vi "FileDialogAsynch.vi"(0 "start path":path=path "", 1 "default name":string, 2 "File dialog event":T1, 5 "pattern (all files)":string, 7 "pattern label":string, 9 "selection mode":T2(ring)=enum."new or existing file", 11 "error in":errorcluster, 12 "button label":string, 13 "prompt":string) -> (15 "error out":errorcluster)   [LabVIEW 2025]
uses:
  FileDialogEvent.ctl
  FileDialogResult.ctl
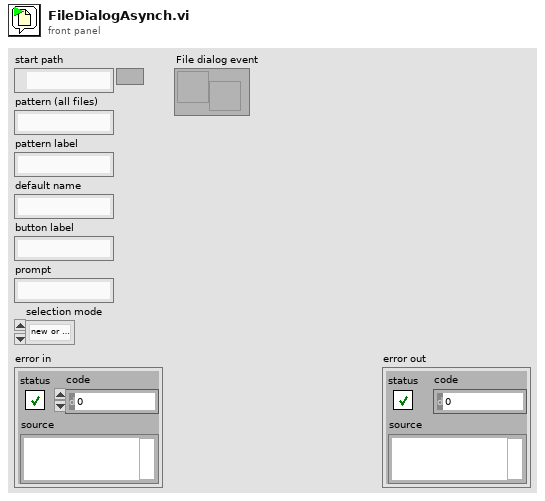
[diagram p1: front panel]
types:
  T1 = typedef "FileDialogEvent.ctl" = refnum<user-event>
  T2 = enum32{"existing file", "new file", "new or existing file", "existing dir", "new dir", "new or existing dir", "existing file (use LLBs)", "new file (use LLBs)", "new or existing file (use LLBs)", "new or existing file or directory (use LLBs)", "existing dir (use LLBs)", "new dir (use LLBs)", "new or existing dir (use LLBs)", "existing file or dir", "new file or dir", "new or existing file or dir", "existing file or dir (use LLBs)", "new file or dir (use LLBs)", "multi-select", "multi-select (use LLBs)"}
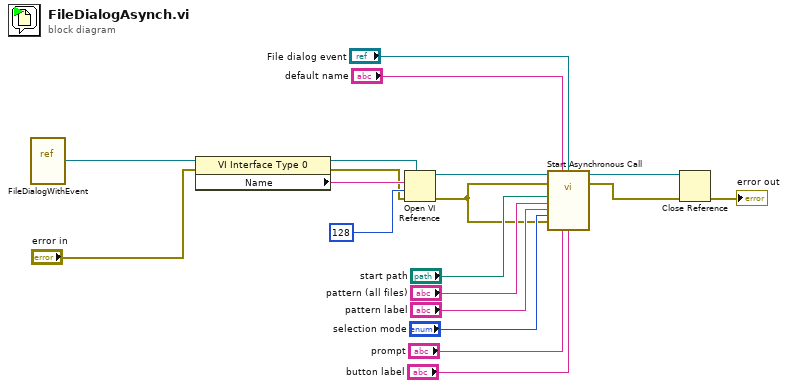
[diagram p0: block diagram]
diagram:
  n1 = vi-ref "FileDialogWithEvent.vi"() -> (w15:refnum<vi>)
  n2 = property class="VI Interface Type 0"(reference=w15, error in="error in") -> (reference out=w1:refnum<vi>, error out=w13:errorcluster, "Name"=w19:string)
  n3 = Open VI Reference(type specifier VI Refnum (for type only)=w1, vi path=w19, options=128, error in (no error)=w13) -> (vi reference=w14:refnum<vi>, error out=w7:errorcluster)  [unwired: 2 in]
  n4 = call-by-ref "Start Asynchronous Call"(reference=w14, error in=w7, "start path"="start path", "default name"="default name", "File dialog event"="File dialog event", "pattern (all files)"="pattern (all files)", "pattern label"="pattern label", "selection mode"="selection mode", "error in"=w7, "prompt"="prompt", "button label"="button label") -> (reference out=w18:refnum<vi>, error out=w17:errorcluster)  [unwired: 5 in, 2 out]
  n5 = Close Reference(reference=w18, error in (no error)=w17) -> (error out=→"error out":errorcluster)
